vi "P11_RunAsyncCloseRef.vi"(11 "Inputs":string[](array[string])) -> (2 "Output/Failure":string, 3 "CLI Process Return Code":i32)   [LabVIEW 2026]
doc: "Slice 1.1 probe: Open VI Reference, Run VI async, read state, Close Reference, Open VI Reference again, read state, close."
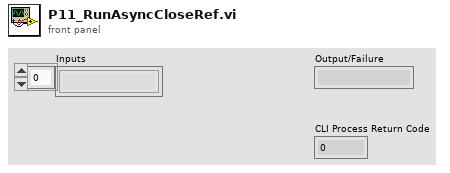
[diagram p1: front panel]
types:
  T1 = enum32{"Bad", "Idle", "Run top level", "Running"}
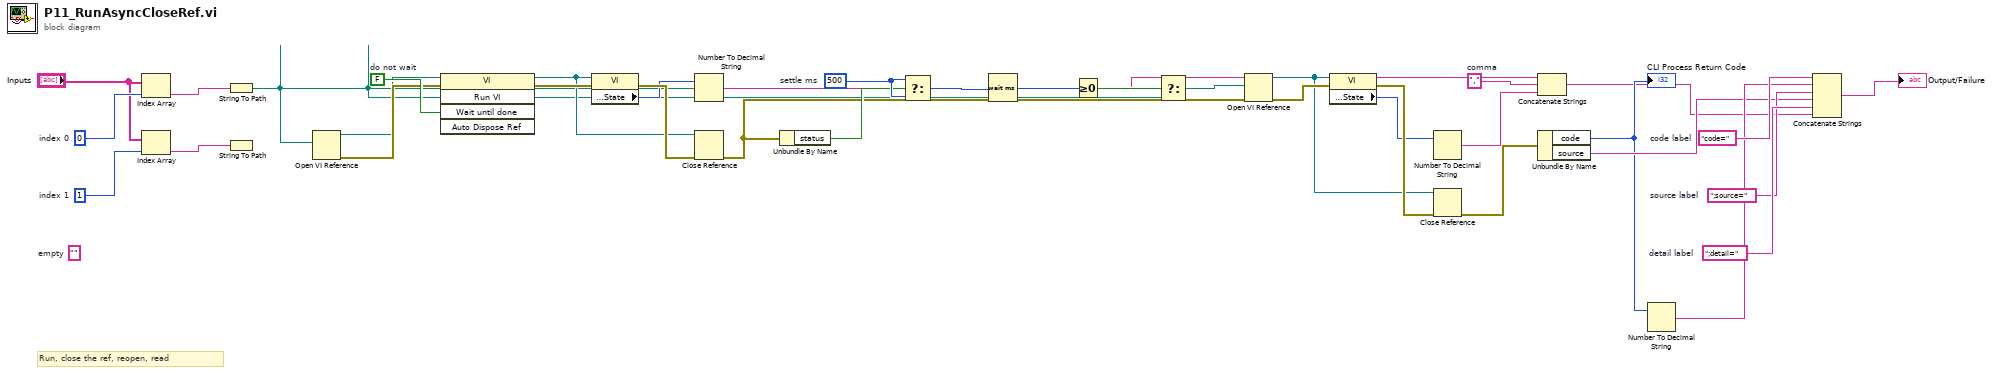
[diagram p0: block diagram]
diagram:
  w35 = ";detail="  # detail label
  w34 = ";source="  # source label
  w33 = "code="  # code label
  w18 = u32 500  # settle ms
  w10 = ","  # comma
  w9 = FALSE  # do not wait
  (unwired) ""  # empty
  w3 = 1  # index 1
  w2 = 0  # index 0
  # "Run, close the ref, reopen, read"
  n1 = Index Array(array="Inputs", index=w2) -> (element=w4:string)
  n2 = Index Array(array="Inputs", index=w3) -> (element=w5:string)
  n3 = String To Path(string=w4) -> (path=w6:path)
  n4 = String To Path(string=w5) -> ()  [unwired: 1 out]
  n5 = Open VI Reference(vi path=w6) -> (vi reference=w7:refnum<vi>, error out=w8:errorcluster)  [unwired: 5 in]
  n6 = invoke class="VI" method="Run VI"(reference=w7, error in=w8, "Wait until done"=w9) -> (reference out=w11:refnum<vi>, error out=w12:errorcluster)  [unwired: 2 in, 3 out]
  n7 = property class="VI"(reference=w11, error in=w12) -> (error out=w14:errorcluster, "Execution:State"=w13:T1)  [unwired: 1 out]
  n8 = Number To Decimal String(number=w13) -> (decimal integer string=w15:string)  [unwired: 1 in]
  n9 = Close Reference(reference=w11, error in (no error)=w14) -> (error out=w16:errorcluster)
  n10 = Unbundle By Name(w16) -> ("status"=w17:bool)
  n11 = Select(t=w18, s=w17, f=w18) -> (s? t:f=w19:u32)
  n12 = Wait (ms)(milliseconds to wait=w19) -> (millisecond timer value=w20:u32)
  n13 = Greater Or Equal To 0?(x=w20) -> (x >= 0?=w21:bool)
  n14 = Select(t=w6, s=w21, f=w6) -> (s? t:f=w22:path)
  n15 = Open VI Reference(vi path=w22, error in (no error)=w16) -> (vi reference=w23:refnum<vi>, error out=w24:errorcluster)  [unwired: 4 in]
  n16 = property class="VI"(reference=w23, error in=w24) -> (error out=w26:errorcluster, "Execution:State"=w25:T1)  [unwired: 1 out]
  n17 = Number To Decimal String(number=w25) -> (decimal integer string=w27:string)  [unwired: 1 in]
  n18 = Close Reference(reference=w23, error in (no error)=w26) -> (error out=w29:errorcluster)
  n19 = Concatenate Strings(w15, w10, w27) -> (w28:string)
  n20 = Unbundle By Name(w29) -> ("code"=w30:i32, "source"=w31:string)
  "CLI Process Return Code" <- w30
  n21 = Number To Decimal String(number=w30) -> (decimal integer string=w32:string)  [unwired: 1 in]
  n22 = Concatenate Strings(w33, w32, w34, w31, w35, w28) -> (→"Output/Failure":string)
